vi "Test Gamma and CLAHE.vi"() -> ()   [LabVIEW 2017, in "Image Processing Library.lvlib"]
uses:
  Image Processing Library.lvlib
panel:
  out "Image Gamma + CLAHE":picture
  out "Image CLAHE":picture
  out "Image Gamma":picture
  out "Image In":picture
  out "error out":errorcluster
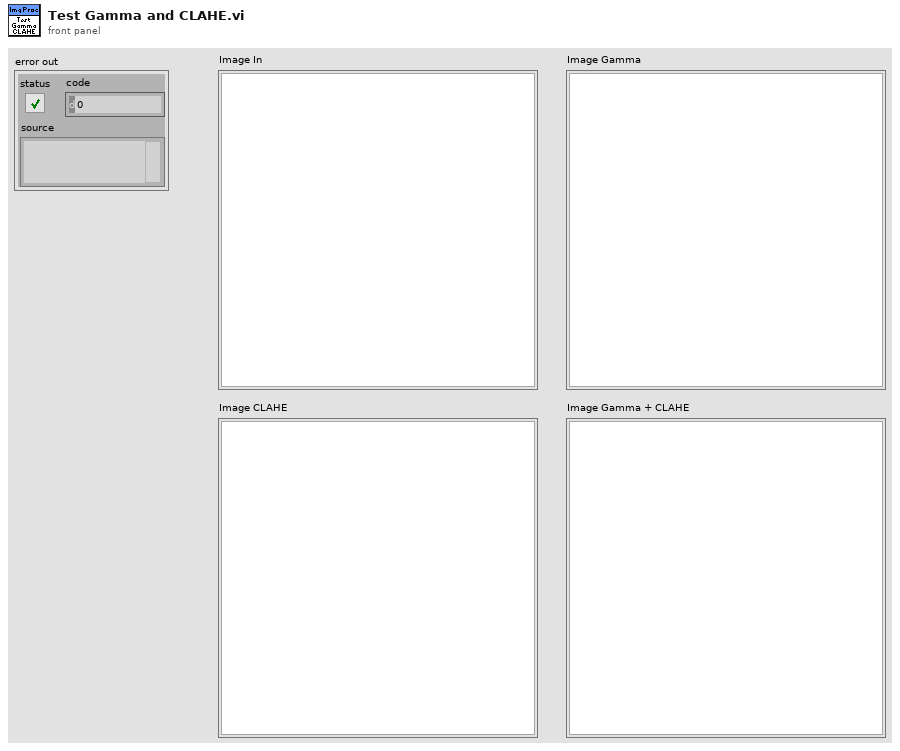
[diagram p1: front panel]
types:
  T1 = typedef "imagedata.ctl" = cluster{"image type":i32, "image depth":i32, "image":u8[], "mask":u8[], "colors":u32[], "Rectangle":cluster{"left":i16, "top":i16, "right":i16, "bottom":i16}}
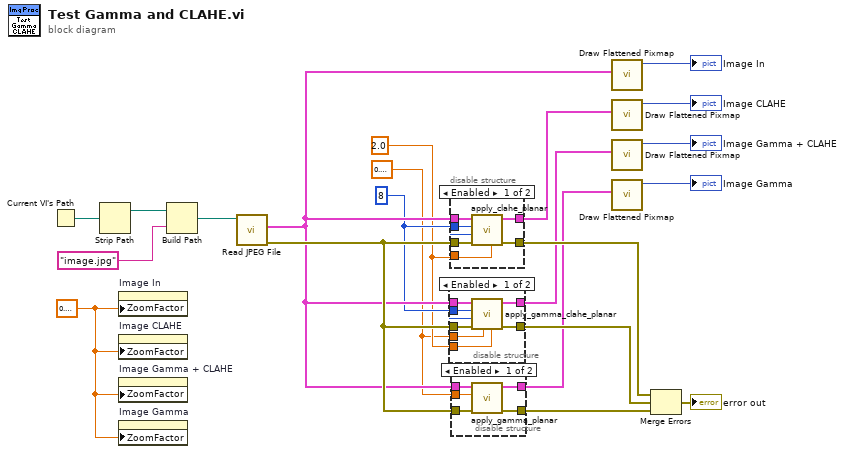
[diagram p0: block diagram]
diagram:
  w2 = sgl 2.0 ("clip_limit")
  w1 = sgl 0.9 ("gamma_value")
  w3 = 8 ("tile_grid_w")
  w4 = sgl 0.3 ("Zoom Factor")
  n1 = Current VI's Path() -> (path=w20:path)
  n2 = Strip Path(path=w20) -> (stripped path=w19:path)  [unwired: 1 out]
  n3 = property on="Image In" class="Pict"("ZoomFactor"=w4) -> ()  [unwired: 2 in, 2 out]
  n4 = property on="Image CLAHE" class="Pict"("ZoomFactor"=w4) -> ()  [unwired: 2 in, 2 out]
  n5 = property on="Image Gamma + CLAHE" class="Pict"("ZoomFactor"=w4) -> ()  [unwired: 2 in, 2 out]
  n6 = property on="Image Gamma" class="Pict"("ZoomFactor"=w4) -> ()  [unwired: 2 in, 2 out]
  n7 = Build Path(base path=w19, name or relative path="image.jpg") -> (appended path=w18:path)
  n8 = call <vilib>:"Read JPEG File.vi"("path to JPEG file"=w18) -> ("error out"=w17:errorcluster, "image data"=w12:T1)  [unwired: 8 in, 1 out]
  n9 = disable-structure shown="Enabled" {
    disable-tunnel: w17 -> [w28 w30]
    disable-tunnel: [w27 w30] -> w15
    disable-tunnel: w12 -> [w26 w29]
    disable-tunnel: [w25 w29] -> w6
    disable-tunnel: w3 -> [w24 _]
    disable-tunnel: w2 -> [w23 _]
    disable-tunnel: w1 -> [w22 _]
    frame Enabled {
      n10 = call "apply_gamma_clahe_planar.vi"("clip_limit"=w23, "gamma_value"=w22, "error in (no error)"=w28, "tile_grid_h"=w24, "tile_grid_w"=w24, "image in"=w26) -> ("error out"=w27:errorcluster, "image out"=w25:T1)  [unwired: 4 in]
    }
    frame Disabled {
    }
  }
  n11 = disable-structure shown="Enabled" {
    disable-tunnel: w17 -> [w36 w38]
    disable-tunnel: [w35 w38] -> w16
    disable-tunnel: w12 -> [w34 w37]
    disable-tunnel: [w33 w37] -> w10
    disable-tunnel: w3 -> [w32 _]
    disable-tunnel: w2 -> [w31 _]
    frame Enabled {
      n12 = call "apply_clahe_planar.vi"("clip_limit"=w31, "error in (no error)"=w36, "tile_grid_h"=w32, "tile_grid_w"=w32, "image in"=w34) -> ("error out"=w35:errorcluster, "image out"=w33:T1)  [unwired: 5 in]
    }
    frame Disabled {
    }
  }
  n13 = disable-structure shown="Enabled" {
    disable-tunnel: w17 -> [w43 w45]
    disable-tunnel: [w42 w45] -> w14
    disable-tunnel: w12 -> [w41 w44]
    disable-tunnel: [w40 w44] -> w5
    disable-tunnel: w1 -> [w39 _]
    frame Enabled {
      n14 = call "apply_gamma_planar.vi"("error in (no error)"=w43, "gamma_value"=w39, "image in"=w41) -> ("error out"=w42:errorcluster, "image out"=w40:T1)  [unwired: 7 in]
    }
    frame Disabled {
    }
  }
  n15 = call <vilib>:"Draw Flattened Pixmap.vi"("image data"=w12) -> ("new picture"=→"Image In":picture)  [unwired: 8 in]
  n16 = call <vilib>:"Draw Flattened Pixmap.vi"("image data"=w10) -> ("new picture"=→"Image CLAHE":picture)  [unwired: 8 in]
  n17 = call <vilib>:"Draw Flattened Pixmap.vi"("image data"=w6) -> ("new picture"=→"Image Gamma + CLAHE":picture)  [unwired: 8 in]
  n18 = call <vilib>:"Draw Flattened Pixmap.vi"("image data"=w5) -> ("new picture"=→"Image Gamma":picture)  [unwired: 8 in]
  n19 = Merge Errors(w16, w15, w14) -> (→"error out":errorcluster)
